vi "lvmcp_caseselector.vi"() -> ()   [LabVIEW 2015]
panel:
  out "error out":errorcluster
  out "UID":i32
  in  "reference":refnum<vi>
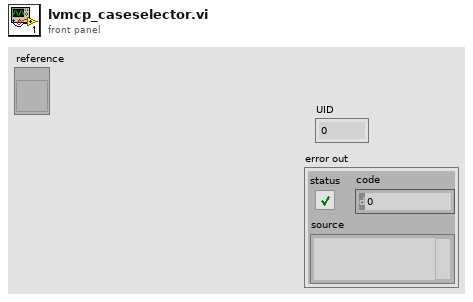
[diagram p1: front panel]
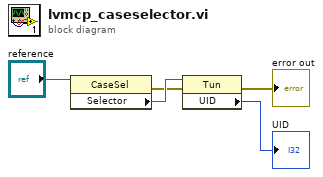
[diagram p0: block diagram]
diagram:
  n1 = property class="CaseSel"(reference="reference") -> (error out=w3:errorcluster, "Selector"=w4:refnum<vi>)  [unwired: 1 in, 1 out]
  n2 = property class="Tun"(reference=w4, error in=w3) -> (error out=→"error out":errorcluster, "UID"=→"UID":i32)  [unwired: 1 out]
